vi "ALL MCS Registers.vi"() -> ()   [LabVIEW 2025]
panel:
  in  "ALL MCS and Chiller":cluster{"Array":string[][]}[](array[cluster])
  out "Chiller Right":string[][](array[string])
  out "Chiller REf":string[][](array[string])
  out "Chiller Left":string[][](array[string])
  out "MCS Tree":string[][](array[string])
  out "MCS Ref":string[][](array[string])
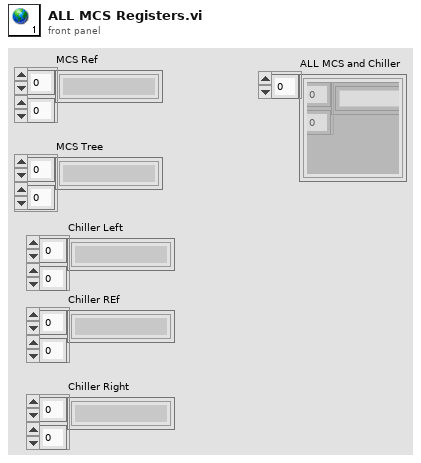
[diagram p1: front panel]
diagram:
